vi "D_Open.vi"(8 "error in (no error)":errorcluster) -> (0 "error out":errorcluster, 2 "bIDList":u8[](array[numeric]), 3 "DevNum":i32)   [LabVIEW 2014]
uses:
  LabVIEW2018/hpkSLMdaLV.dll
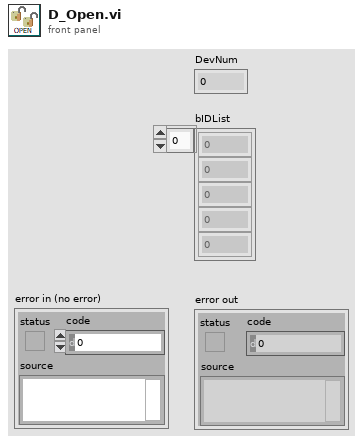
[diagram p1: front panel]
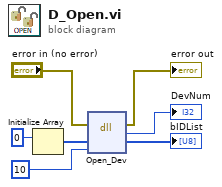
[diagram p0: block diagram]
diagram:
  n1 = Initialize Array(u8 0 ("要素")) -> (w5:u8[])  [unwired: 1 in]
  n2 = dll-call lib="C:/Users/hs5921/Desktop/LabVIEW2018/hpkSLMdaLV.dll" fn="Open_Dev"(error in="error in (no error)", "bIDList"=w5, "bIDSize"=10) -> (error out=→"error out":errorcluster, "返り値タイプ"=→"DevNum":i32, "bIDList"=→"bIDList":u8[])  [unwired: 3 in, 1 out]
